vi "RPC Method ThermalChamberController UpdateHeaterState.vi"(8 "error in (no error)":errorcluster, 11 "gRPC service in":refnum<class "ThermalChamberController.lvclass">) -> (0 "error out":errorcluster, 3 "gRPC service out":refnum<class "ThermalChamberController.lvclass">)   [LabVIEW 2020, in "thermal-chamber-controller_server.lvlib" / "ThermalChamberController.lvclass"]
uses:
  ThermalChamberController.lvclass
  ThermalChamberController.lvclass/ThermalChamberController.ctl
  RPC Messages/lv_python_grpc_webui_demo_v1_Empty.ctl
  Program Files (x86)/National Instruments/LabVIEW 2020/examples/DQMH Consortium/DQMH Fundamentals - Thermal Chamber/Libraries/Thermal Chamber Controller_DQMH/Heater State--enum.ctl
  Program Files (x86)/National Instruments/LabVIEW 2020/examples/DQMH Consortium/DQMH Fundamentals - Thermal Chamber/Libraries/Thermal Chamber Controller_DQMH/Thermal Chamber Controller_DQMH.lvlib
  thermal-chamber-controller_server.lvlib
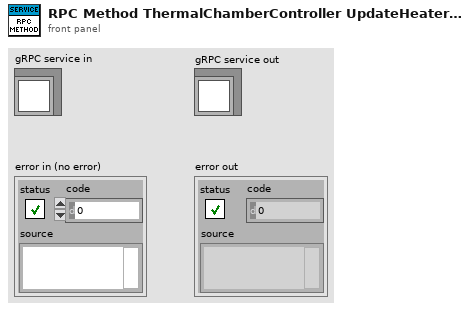
[diagram p1: front panel]
types:
  T1 = typedef "thermal-chamber-controller_server.lvlib/lv_python_grpc_webui_demo_v1_Empty.ctl" = cluster{"void":string}
  T2 = typedef "Thermal Chamber Controller_DQMH.lvlib/Heater State--enum.ctl" = enum16{"Heater Enabled", "Heater Disabled"}
  T3 = typedef "thermal-chamber-controller_server.lvlib/ThermalChamberController.lvclass/Server Internal UEs.ctl" = cluster{"ThermalChamberController StartModule Internal UE":refnum<user-event>, "ThermalChamberController ShowModulePanel Internal UE":refnum<user-event>, "ThermalChamberController HideModulePanel Internal UE":refnum<user-event>, "ThermalChamberController StopModule Internal UE":refnum<user-event>, "ThermalChamberController UpdateSetPoint Internal UE":refnum<user-event>, "ThermalChamberController UpdateRampRate Internal UE":refnum<user-event>, "ThermalChamberController UpdateHeaterState Internal UE":refnum<user-event>, "ThermalChamberController SubscribeChamberStatusUpdated Internal UE":refnum<user-event>, "ThermalChamberController SubscribeSetPointUpdated Internal UE":refnum<user-event>, "ThermalChamberController SubscribeRampRateUpdated Internal UE":refnum<user-event>, "ThermalChamberController SubscribeHeaterStateUpdated Internal UE":refnum<user-event>}
  T4 = typedef "thermal-chamber-controller_server.lvlib/ThermalChamberController.lvclass/Server gRPC UEs.ctl" = cluster{"ThermalChamberController StartModule gRPC UE":refnum<user-event>, "ThermalChamberController ShowModulePanel gRPC UE":refnum<user-event>, "ThermalChamberController HideModulePanel gRPC UE":refnum<user-event>, "ThermalChamberController StopModule gRPC UE":refnum<user-event>, "ThermalChamberController UpdateSetPoint gRPC UE":refnum<user-event>, "ThermalChamberController UpdateRampRate gRPC UE":refnum<user-event>, "ThermalChamberController UpdateHeaterState gRPC UE":refnum<user-event>, "ThermalChamberController SubscribeChamberStatusUpdated gRPC UE":refnum<user-event>, "ThermalChamberController SubscribeSetPointUpdated gRPC UE":refnum<user-event>, "ThermalChamberController SubscribeRampRateUpdated gRPC UE":refnum<user-event>, "ThermalChamberController SubscribeHeaterStateUpdated gRPC UE":refnum<user-event>}
  T5 = typedef "grpc-lvsupport-release.lvlib/grpcId.ctl" = u64
  T6 = typedef "thermal-chamber-controller_server.lvlib/lv_python_grpc_webui_demo_v1_UpdateHeaterStateRequest.ctl" = cluster{"heater_state":T7}
  T7 = typedef "thermal-chamber-controller_server.lvlib/lv_python_grpc_webui_demo_v1_HeaterState.ctl" = enum32{"HEATER_ENABLED", "HEATER_DISABLED"}
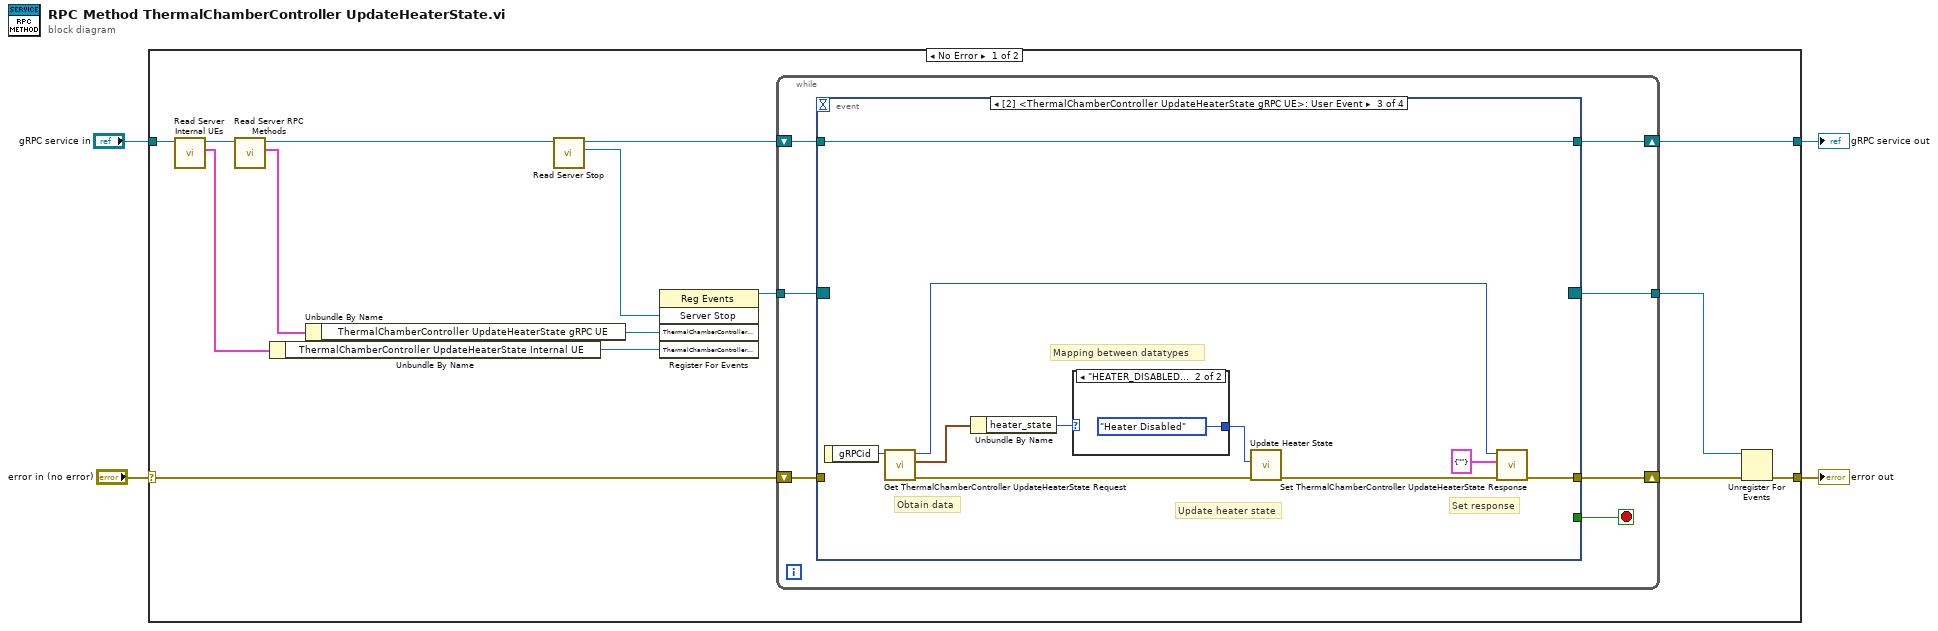
[diagram p0: block diagram]
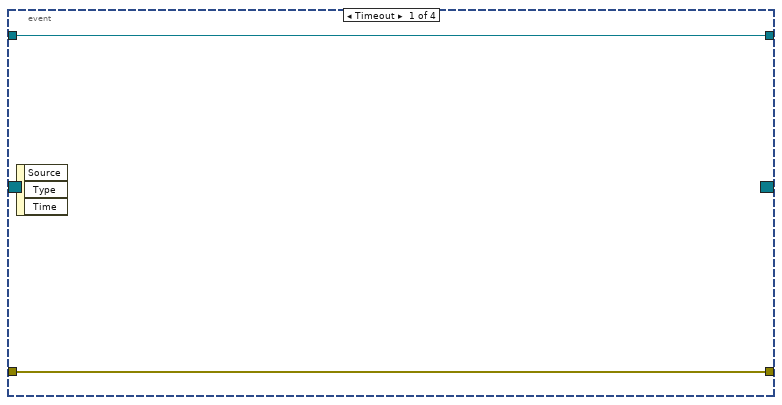
[diagram p2: hidden frame]
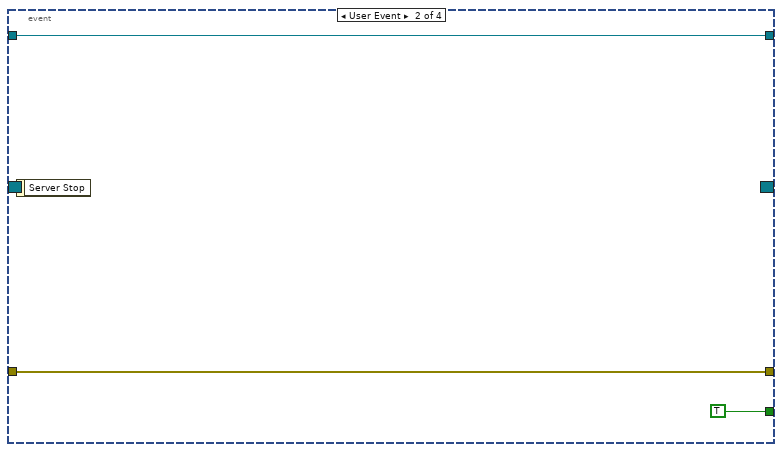
[diagram p3: hidden frame]
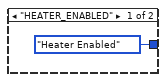
[diagram p4: hidden frame]
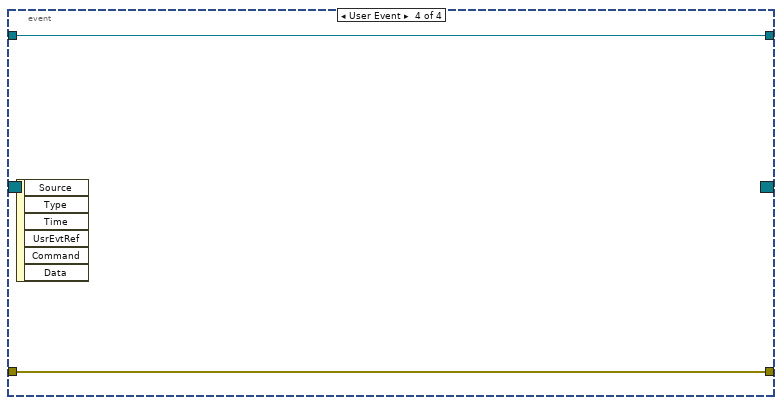
[diagram p5: hidden frame]
diagram:
  n1 = case shown="No Error" "error in (no error)" {
    selector: "error in (no error)" -> [w15 w47]
    tunnel: [w13 w47] -> w3
    tunnel: "gRPC service in" -> [w17 w46]
    tunnel: [w5 w46] -> w1
    frame No Error {
      n2 = call "Read Server Internal UEs.vi"("gRPC service in"=w17) -> ("Server Internal UEs"=w9:T3, "gRPC service out"=w16:refnum<class "ThermalChamberController.lvclass">)  [unwired: 8 in, 1 out]
      n3 = call "Read Server RPC Methods.vi"("gRPC service in"=w16) -> ("Server RPC Methods"=w11:T4, "gRPC service out"=w6:refnum<class "ThermalChamberController.lvclass">)  [unwired: 8 in, 1 out]
      n4 = Unbundle By Name ("Unbundle Internal UE")(w9) -> ("ThermalChamberController UpdateHeaterState Internal UE"=w8:refnum<user-event>)
      n5 = Unbundle By Name ("Unbundle gRPC UE")(w11) -> ("ThermalChamberController UpdateHeaterState gRPC UE"=w10:refnum<user-event>)
      n6 = call-dynamic "Read Server Stop.vi"("gRPC service in"=w6) -> ("Server Stop"=w19:refnum<user-event>, "gRPC service out"=w7:refnum<class "ThermalChamberController.lvclass">)  [unwired: 8 in, 1 out]
      n7 = register-events(w19, w10, w8) -> (reference out=w18:refnum<event-registration>)  [unwired: 2 in, 1 out]
      n8 = while {
        tunnel: w18 -> [w26]
        tunnel: [w22] -> w12
        shift-right: [w23] -> w14
        shift-left: w15 -> [w24]
        shift-right: [w20] -> w5
        shift-left: w7 -> [w21]
        stop <- w25 stop-if-true
        n9 = event "RPC Method Event Structure" shown="[2] <ThermalChamberController UpdateHeaterState gRPC UE>: User Event" {
          selector: w26 -> [_ _ _ _]
          dyn-events: [_ _ _ _] -> w22
          timeout: _ -> [_ _ _ _]
          tunnel: [_ TRUE _ _] -> w25
          tunnel: w24 -> [w28 w30 _ w45]
          tunnel: [w28 w30 w35 w45] -> w23
          tunnel: w21 -> [w27 w29 w41 w44]
          tunnel: [w27 w29 w41 w44] -> w20
          event Timeout {
            n10 = event-data() -> ()  [unwired: 1 in, 3 out]
          }
          event User Event {
            n11 = event-data() -> ()  [unwired: 1 in, 1 out]
          }
          event User Event {
            # "Mapping between datatypes"
            # "Set response"
            # "Obtain data"
            # "Update heater state"
            n12 = event-data() -> ("gRPCid"=w34:T5)  [unwired: 1 in]
            n13 = call "Get ThermalChamberController UpdateHeaterState Request.vi"("gRPCid"=w34) -> ("error out"=w39:errorcluster, "Message Data"=w40:T6, "gRPCid out"=w37:T5)  [unwired: 8 in]
            n14 = Unbundle By Name(w40) -> ("heater_state"=w33:T7)
            n15 = case shown="\"HEATER_DISABLED\"" w33 {
              tunnel: [Heater_State--enum."Heater Enabled" ("Heater State") Heater_State--enum."Heater Disabled" ("Heater State")] -> w32
              frame "HEATER_ENABLED" {
              }
              frame "HEATER_DISABLED" {
              }
            }
            n16 = call "Update Heater State.vi"("error in"=w39, "Heater State"=w32) -> ("error out"=w38:errorcluster)  [unwired: 9 in]
            n17 = call "Set ThermalChamberController UpdateHeaterState Response.vi"("error in (no error)"=w38, "Message Data"=T1 {"void"=""}, "gRPCid in"=w37) -> ("error out"=w35:errorcluster)  [unwired: 8 in]
          }
          event User Event {
            n18 = event-data() -> ()  [unwired: 1 in, 6 out]
          }
        }
      }
      n19 = Unregister For Events(event registration refnum=w12, error in=w14) -> (error out=w13:errorcluster)
    }
    frame Error {
    }
  }
  "error out" <- w3
  "gRPC service out" <- w1
